vi "ZM-ROOT-launchHwm.vi"(8 "error in (no error)":errorcluster, 11 "ZM-ROOT-root in":refnum<class "ZM-ROOT-root.lvclass">) -> (0 "error out":errorcluster, 3 "ZM-ROOT-root out":refnum<class "ZM-ROOT-root.lvclass">)   [LabVIEW 2020, in "ZM-ROOT-root.lvlib" / "ZM-ROOT-root.lvclass"]
doc: "Launches the hardware manager, called by ZM-ROOT-init after launchCm, with intervalMs = 500 and the simulated hardware, or the bare placeholder hardware (its methods return 5000) when usePlaceholderHardware is set. Stores its enqueuer."
uses:
  ZM-ROOT-root.lvclass
  hardware/ZM-HW-SIM-simulated_hardware/ZM-HW-SIM-simulated_hardware/ZM-HW-SIM-simulated_hardware.lvclass
  hardware/ZM-HW-hardware/ZM-HW-hardware/ZM-HW-hardware.lvclass
  ZM-ROOT-root.lvclass/ZM-ROOT-root.ctl
  ZM-HWM-hardware_manager/ZM-HWM-hardware_manager/ZM-HWM-hardware_manager.lvclass
  <vilib>/ActorFramework/Actor/Actor.lvclass
  ZM-HWM-hardware_manager/ZM-HWM-hardware_manager/ZM-HWM-PRELAUNCH_SETTINGS.ctl
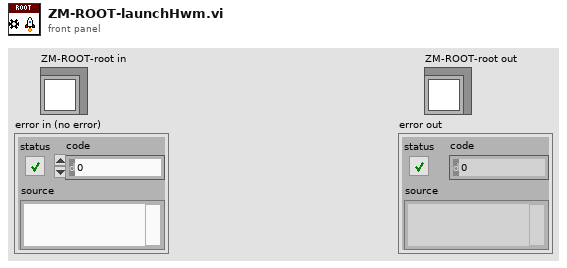
[diagram p1: front panel]
types:
  T1 = typedef "ZM-HWM-hardware_manager.lvlib/ZM-HWM-hardware_manager.lvclass/ZM-HWM-PRELAUNCH_SETTINGS.ctl" = cluster{"hardware":refnum<class "ZM-HW-hardware.lvclass">, "intervalMs":u32}
  T2 = typedef "ZM-ROOT-root.lvlib/ZM-ROOT-root.lvclass/ZM-ROOT-PRELAUNCH_SETTINGS.ctl" = cluster{"outputFolder":path, "usePlaceholderHardware":bool}
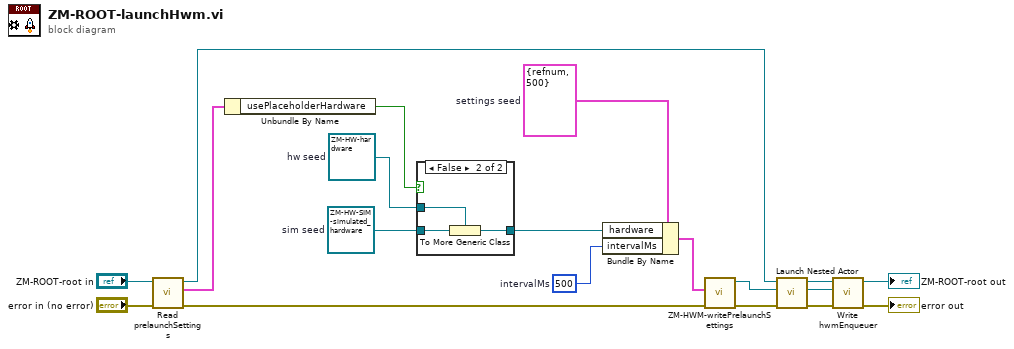
[diagram p0: block diagram]
diagram:
  w12 = u32 500  # intervalMs
  w11 = T1 {"hardware"=refnum, "intervalMs"=500}  # settings seed
  w15 = refnum<class "ZM-HW-hardware.lvclass"> refnum  # hw seed
  w16 = refnum<class "ZM-HW-SIM-simulated_hardware.lvclass"> refnum  # sim seed
  n1 = call "Read prelaunchSettings.vi"("error in (no error)"="error in (no error)", "ZM-ROOT-root in"="ZM-ROOT-root in") -> ("error out"=w9:errorcluster, "ZM-ROOT-PRELAUNCH_SETTINGS"=w17:T2, "ZM-ROOT-root out"=w6:refnum<class "ZM-ROOT-root.lvclass">)  [unwired: 7 in]
  n2 = Unbundle By Name(w17) -> ("usePlaceholderHardware"=w14:bool)
  n3 = case shown="False" w14 {
    tunnel: w16 -> [_ w23]
    tunnel: w15 -> [w20 w22]
    tunnel: [w20 w21] -> w13
    frame True {
    }
    frame False {
      n4 = To More Generic Class(target class=w22, reference=w23) -> (generic class reference=w21:refnum<class "ZM-HW-hardware.lvclass">)
    }
  }
  n5 = Bundle By Name(cluster=w11, "hardware"=w13, "intervalMs"=w12) -> (w10:T1)
  n6 = call "ZM-HWM-writePrelaunchSettings.vi"("error in (no error)"=w9, "settings"=w10) -> ("error out"=w7:errorcluster, "ZM-HWM-hardware_manager out"=w8:refnum<class "ZM-HWM-hardware_manager.lvclass">)  [unwired: 8 in]
  n7 = call <vilib>:"Launch Nested Actor.vi"("error in (no error)"=w7, "Nested Actor"=w8, "Caller Actor in"=w6) -> ("error out"=w5:errorcluster, "Nested Actor's Enqueuer"=w3:refnum<class "Message Enqueuer.lvclass">, "Caller Actor out"=w4:refnum<class "ZM-ROOT-root.lvclass">)  [unwired: 6 in]
  n8 = call "Write hwmEnqueuer.vi"("error in (no error)"=w5, "Actor Framework:Message Enqueuer"=w3, "ZM-ROOT-root in"=w4) -> ("error out"=→"error out":errorcluster, "ZM-ROOT-root out"=→"ZM-ROOT-root out":refnum<class "ZM-ROOT-root.lvclass">)  [unwired: 7 in]
